vi "drive-auto.vi"() -> ()   [LabVIEW 2018]
doc: "This VI is called for each TeleOp packet received from the DS where the robot is not disabled. It is often used to read from the joysticks and update I/O or to update setpoints for timed control loops. It should complete and return within 20 milliseconds or it may miss DS packets."
uses:
  <vilib>/Rock Robotics/WPI/Solenoid/WPI_SolenoidValue.ctl
  <vilib>/Rock Robotics/WPI/ThirdParty/Phoenix-LabVIEW/Motor Controller/Controls/CTRE_Phoenix_MotorControl_ControlMode.ctl
  069bde93-6a50-4702-a448-63a100da85ba.vi
  93fe4f39-d887-44e8-b42b-40b0db67de57.vi
  <vilib>/Rock Robotics/WPI/Utilities/WPI_GetSetVariantRefNum.vi
  <vilib>/Rock Robotics/Network Tables/NT Write Boolean Array.vi
  <vilib>/Rock Robotics/Network Tables/NT Write Numeric Array.vi
  Robot Global Data.vi
  <vilib>/Rock Robotics/WPI/Solenoid/WPI_SolenoidSetEnum.vi
  <vilib>/Rock Robotics/WPI/ThirdParty/Phoenix-LabVIEW/Motor Controller/Get/CTRE_Phoenix_MotorController_GetSelectedSensorData.vi
  <vilib>/Rock Robotics/WPI/ThirdParty/Phoenix-LabVIEW/Motor Controller/Get/CTRE_Phoenix_MotorController_GetOutputCurrent_Enhanced.vi
panel:
  out "Level":string="Low"
  out "GamePiece":string="Hatch"
  out "Output Voltage 4":dbl
  out "Output Voltage 3":dbl
  out "Output Voltage 2":dbl
  out "Output Voltage":dbl
  out "wrist sensor":i32
  out "Arm sensor":i32
  out "x output 2":dbl
  out "y output 2":dbl
  # "left"
  # "RIGHT"
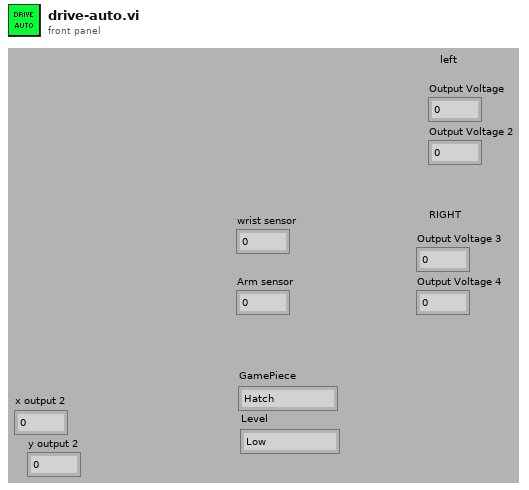
[diagram p1: front panel]
types:
  T1 = typedef "WPI_SolenoidValue.ctl" = enum16{"Off", "On", "Forward", "Reverse"}
  T2 = typedef "WPI_JoystickDevRef.ctl" = cluster{"Device":T3}
  T3 = typedef "WPI_JoystickDeviceEnum.ctl" = enum16{"USB 0", "USB 1", "USB 2", "USB 3", "USB 4", "USB 5"}
  T4 = typedef "WPI_RobotDriveDevRef.ctl" = cluster{"DevStatus":errorcluster, "Motors[]":T5[], "Square Inputs":bool, "Max Output":dbl}
  T5 = typedef "WPI_MotorControlDeviceRef.ctl" = cluster{"DeviceStatus":errorcluster, "Type":T6, "PWM":cluster{"PWM Channel":T7, "DeadBand":T8}, "CAN":cluster{"Device Number":u8, "SetOutput VI Ref":variant, "GetOutput VI Ref":variant, "Enable VI Ref":variant, "Disable VI Ref":variant, "Data":variant}, "Invert":bool, "DIO PWM":cluster{"PWM \"Enable\" Channel":T7, "DIOChannel":T9, "PWM Rate":dbl}}
  T6 = typedef "WPI_MotorControlType.ctl" = enum16{"PWM", "CAN", "DIO PWM"}
  T7 = typedef "FPGA_DIOPWMChannel.ctl" = enum8{"PWM 0", "PWM 1", "PWM 2", "PWM 3", "PWM 4", "PWM 5", "PWM 6", "PWM 7", "PWM 8", "PWM 9", "PWM MXP 0", "PWM MXP 1", "PWM MXP 2", "PWM MXP 3", "PWM MXP 4", "PWM MXP 5", "PWM MXP 6", "PWM MXP 7", "PWM MXP 8", "PWM MXP 9", "Invalid"}
  T8 = typedef "WPI_PWMDeadband.ctl" = cluster{"Name":string, "maxPositivePwm":i32, "minPositivePwm":i32, "centerPwm":i32, "maxNegativePwm":i32, "minNegativePwm":i32, "angularRange":u16}
  T9 = typedef "FPGA_DIOChannel.ctl" = enum8{"DIO 0", "DIO 1", "DIO 2", "DIO 3", "DIO 4", "DIO 5", "DIO 6", "DIO 7", "DIO 8", "DIO 9", "DIO MXP 0", "DIO MXP 1", "DIO MXP 2", "DIO MXP 3", "DIO MXP 4", "DIO MXP 5", "DIO MXP 6", "DIO MXP 7", "DIO MXP 8", "DIO MXP 9", "DIO MXP 10", "DIO MXP 11", "DIO MXP 12", "DIO MXP 13", "DIO MXP 14", "DIO MXP 15", "SPI Port CS1", "SPI Port CS2", "SPI Port CS3", "SPI Port MISO", "SPI Port MOSI", "Invalid"}
  T10 = typedef "WPI_SolenoidDevRef.ctl" = cluster{"DevStatus":errorcluster, "Pneumatics Control Module":u8, "Forward Solenoid Channel":T11, "Reverse Solenoid Channel":T11}
  T11 = typedef "WPI_SolenoidChannel.ctl" = enum8{"Solenoid 0", "Solenoid 1", "Solenoid 2", "Solenoid 3", "Solenoid 4", "Solenoid 5", "Solenoid 6", "Solenoid 7", "Invalid"}
  T12 = typedef "CTRE_Phoenix_MotorControl_ControlMode.ctl" = u16
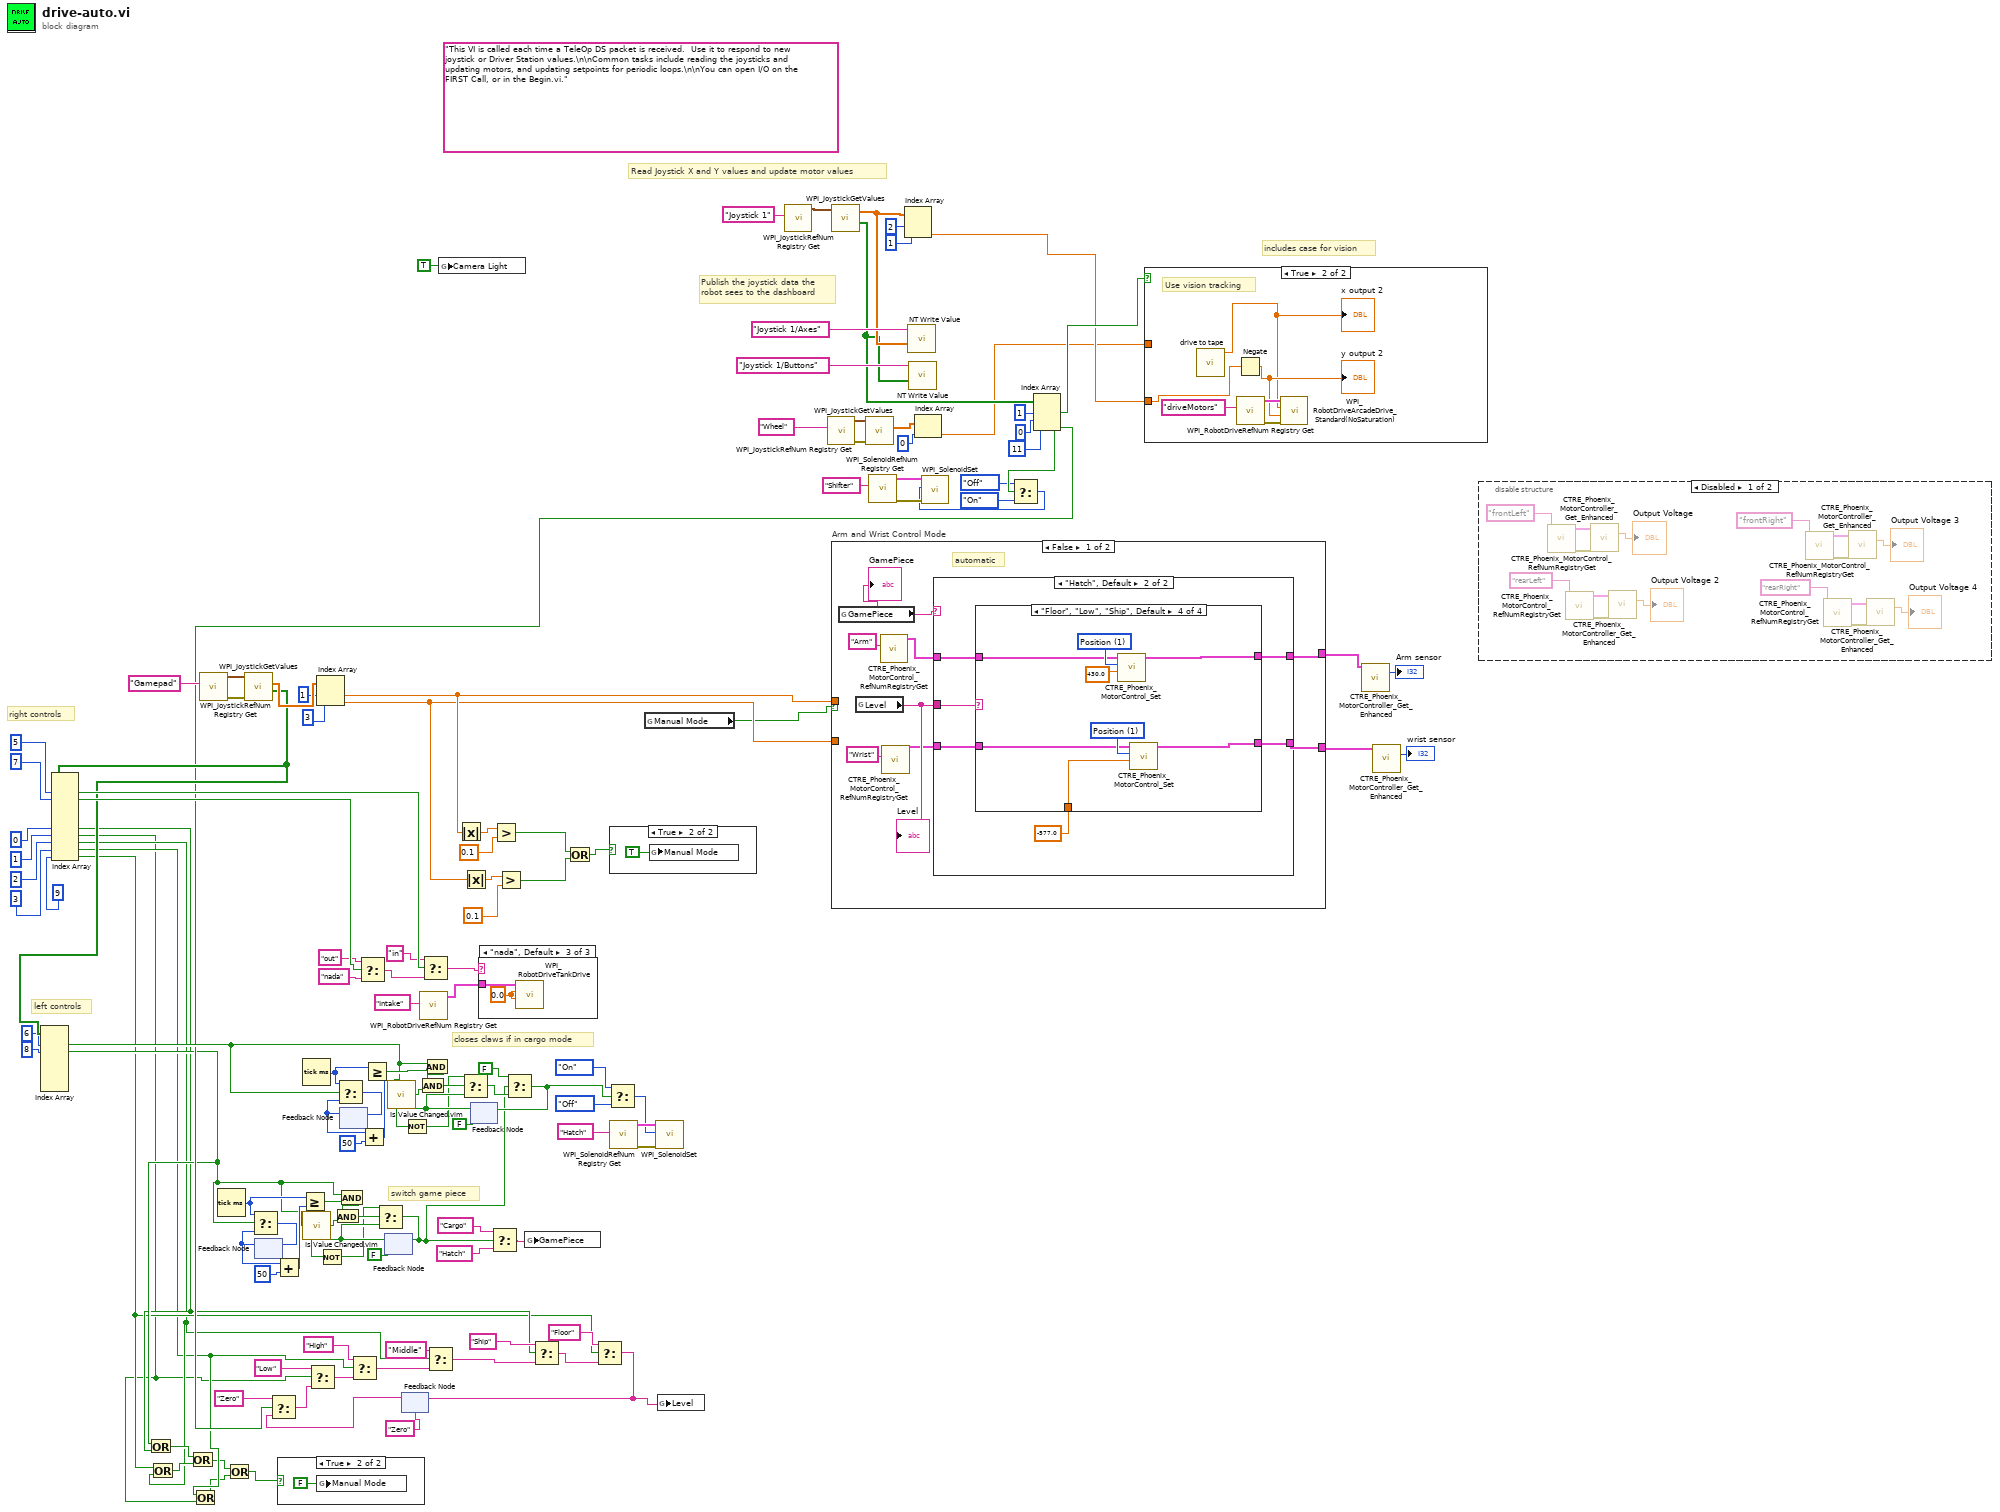
[diagram p0: block diagram]
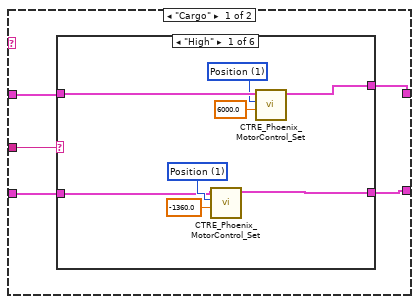
[diagram p5: hidden frame]
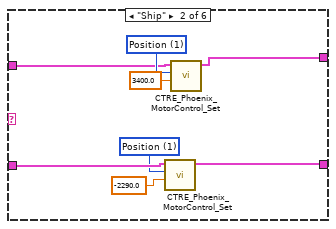
[diagram p6: hidden frame]
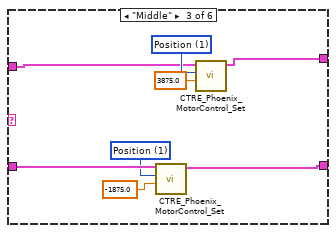
[diagram p7: hidden frame]
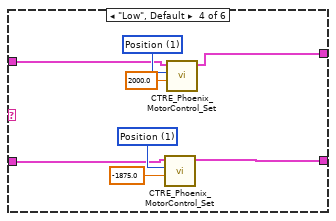
[diagram p8: hidden frame]
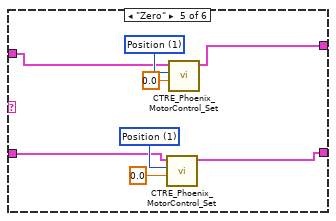
[diagram p9: hidden frame]
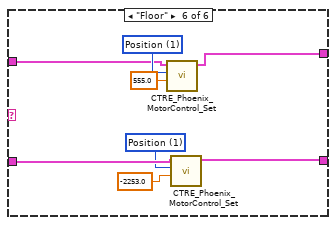
[diagram p10: hidden frame]
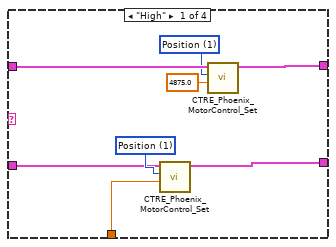
[diagram p11: hidden frame]
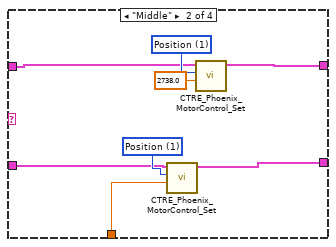
[diagram p12: hidden frame]
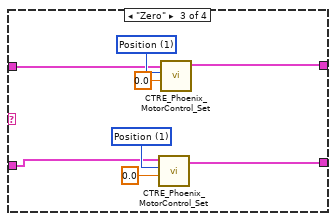
[diagram p13: hidden frame]
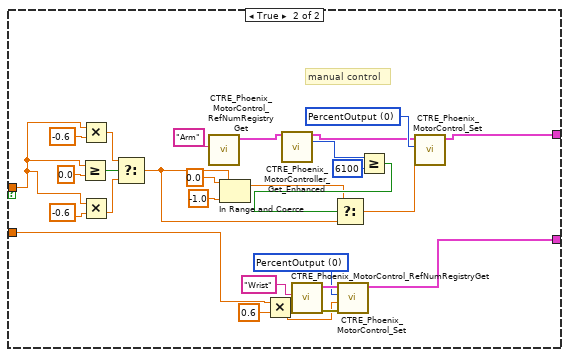
[diagram p14: hidden frame]
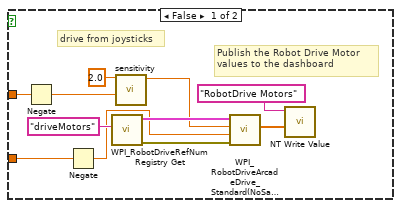
[diagram p15: hidden frame]
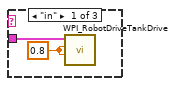
[diagram p16: hidden frame]
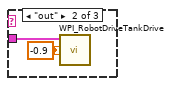
[diagram p17: hidden frame]
diagram:
  (unwired) "This VI is called each time a TeleOp DS packet is received.  Use it to respond to new joystick or Driver Station values.\n\nCommon tasks include reading the joysticks and updating motors, and updating setpoints for periodic loops.\n\nYou can open I/O on the FIRST Call, or in the Begin.vi."
  # "closes claws if in cargo mode"
  # "switch game piece"
  # "left controls"
  # "right controls"
  # "includes case for vision"
  # "Publish the joystick data the\nrobot sees to the dashboard"
  # "Read Joystick X and Y values and update motor values"
  n1 = call <vilib>:"WPI_JoystickRefNum Registry Get.vi"("refnum name"="Gamepad") -> ("error out"=w112:errorcluster, "JoystickDevRef"=w115:T2)  [unwired: 1 in, 8 out]
  n2 = Tick Count (ms)() -> (millisecond timer value=w62:u32)
  n3 = call <vilib>:"WPI_JoystickGetValues.vi"("error in (no error)"=w112, "JoystickDevRef"=w115) -> ("Buttons"=w36:bool[], "Axes"=w114:dbl[])  [unwired: 5 in, 3 out]
  n4 = Index Array(array=w36, index #1=6 ("index"), index #2=8 ("index")) -> (element #1=w33:bool, element #2=w9:bool)  [unwired: 5 in, 5 out]
  n5 = Index Array(array=w36, index #1=5 ("index"), index #2=7 ("index"), index #6=0 ("index"), index #7=1 ("index"), index #8=2 ("index"), index #9=3 ("index"), index #10=9 ("index")) -> (element #1=w109:bool, element #2=w104:bool, element #6=w8:bool, element #7=w4:bool, element #8=w6:bool, element #9=w5:bool, element #10=w7:bool)  [unwired: 3 in, 3 out]
  n6 = Or(x=w9, y=w8) -> (x .or. y?=w11:bool)
  n7 = Or(x=w7, y=w6) -> (x .or. y?=w10:bool)
  n8 = Or(x=w11, y=w10) -> (x .or. y?=w2:bool)
  n9 = Or(x=w5, y=w4) -> (x .or. y?=w3:bool)
  n10 = Or(x=w2, y=w3) -> (x .or. y?=w1:bool)
  n11 = feedback #1() -> (w53:u32)  [unwired: 1 in]
  n12 = Select(t=w62, s=w9, f=w53) -> (s? t:f=w60:u32)
  n13 = feedback-in #1(w60) -> ()
  n14 = Add(x=w53, y=u32 50) -> (x+y=w61:u32)
  n15 = case shown="True" w1 {
    frame False {
    }
    frame True {
      n16 = global write "Robot Global Data.vi" "Manual Mode"(FALSE) -> ()
    }
  }
  n17 = Greater Or Equal?(x=w62, y=w61) -> (x >= y?=w63:bool)
  n18 = Tick Count (ms)() -> (millisecond timer value=w79:u32)
  n19 = call "Is Value Changed.vim"("value"=w9) -> ("changed or first call?"=w58:bool)
  n20 = Index Array(array=w114, index #1=1 ("index"), index #2=3 ("index")) -> (element #1=w20:dbl, element #2=w15:dbl)
  n21 = And(x=w9, y=w63) -> (x .and. y?=w64:bool)
  n22 = And(x=w64, y=w58) -> (x .and. y?=w57:bool)
  n23 = feedback #2() -> (w70:u32)  [unwired: 1 in]
  n24 = Select(t=w79, s=w33, f=w70) -> (s? t:f=w77:u32)
  n25 = feedback-in #2(w77) -> ()
  n26 = Select(t="out", s=w104, f="nada") -> (s? t:f=w105:string)
  n27 = Add(x=w70, y=u32 50) -> (x+y=w78:u32)
  n28 = Greater Or Equal?(x=w79, y=w78) -> (x >= y?=w80:bool)
  n29 = feedback #3(FALSE) -> (w56:bool)
  n30 = Not(x=w56) -> (.not. x?=w54:bool)
  n31 = Select(t=w54, s=w57, f=w56) -> (s? t:f=w24:bool)
  n32 = feedback-in #3(w24) -> ()
  n33 = call "Is Value Changed.vim"("value"=w33) -> ("changed or first call?"=w75:bool)
  n34 = feedback #4("Zero") -> (w30:string)
  n35 = call <vilib>:"WPI_RobotDriveRefNum Registry Get.vi"("refnum name"="Intake") -> ("RobotDriveDevRef"=w100:T4)  [unwired: 9 in, 1 out]
  n36 = Select(t="in", s=w109, f=w105) -> (s? t:f=w108:string)
  n37 = And(x=w33, y=w80) -> (x .and. y?=w81:bool)
  n38 = And(x=w81, y=w75) -> (x .and. y?=w74:bool)
  n39 = global write "Robot Global Data.vi" "Camera Light"(TRUE ("Camera Light")) -> ()
  n40 = Absolute Value(x=w20) -> (abs(x)=w22:dbl)
  n41 = Absolute Value(x=w15) -> (abs(x)=w18:dbl)
  n42 = feedback #5(FALSE) -> (w73:bool)
  n43 = Not(x=w73) -> (.not. x?=w71:bool)
  n44 = Select(t=w71, s=w74, f=w73) -> (s? t:f=w25:bool)
  n45 = case shown="\"nada\", Default" w108 {
    tunnel: w100 -> [w132 w134 w136]
    frame "in" {
      w133 = 0.8
      n46 = call <vilib>:"WPI_RobotDriveTankDrive.vi"("Right axis value"=w133, "Left axis value"=w133, "RobotDriveDevRef"=w132) -> ()  [unwired: 6 in, 3 out]
    }
    frame "out" {
      w135 = -0.9
      n47 = call <vilib>:"WPI_RobotDriveTankDrive.vi"("Right axis value"=w135, "Left axis value"=w135, "RobotDriveDevRef"=w134) -> ()  [unwired: 6 in, 3 out]
    }
    frame "nada", Default {
      w137 = 0.0
      n48 = call <vilib>:"WPI_RobotDriveTankDrive.vi"("Right axis value"=w137, "Left axis value"=w137, "RobotDriveDevRef"=w136) -> ()  [unwired: 6 in, 3 out]
    }
  }
  n49 = Select(t="Cargo", s=w24, f="Hatch") -> (s? t:f=w66:string)
  n50 = Greater?(x=w22, y=0.1) -> (0:w19:bool)
  n51 = Greater?(x=w18, y=0.1) -> (0:w16:bool)
  n52 = Select(t=FALSE, s=w24, f=w25) -> (s? t:f=w26:bool)
  n53 = feedback-in #5(w26) -> ()
  n54 = global write "Robot Global Data.vi" "GamePiece"(w66) -> ()
  n55 = Or(x=w19, y=w16) -> (x .or. y?=w13:bool)
  n56 = Select(t=WPI_SolenoidValue."On" ("Value"), s=w26, f=WPI_SolenoidValue."Off") -> (s? t:f=w96:T1)
  n57 = case shown="True" w13 {
    frame False {
    }
    frame True {
      n58 = global write "Robot Global Data.vi" "Manual Mode"(TRUE) -> ()
    }
  }
  n59 = call <vilib>:"WPI_SolenoidRefNum Registry Get.vi"("refnum name"="Hatch") -> ("error out"=w99:errorcluster, "SolenoidDevRef"=w98:T10)  [unwired: 9 in]
  n60 = global read "Robot Global Data.vi" "Manual Mode"() -> (w14:bool)
  n61 = call-poly <vilib>:"WPI_SolenoidSet.vi"("error in (no error)"=w99, "Value"=w96, "SolenoidDevRef"=w98) -> ()  [unwired: 7 in, 2 out]
  n62 = call <vilib>:"WPI_JoystickRefNum Registry Get.vi"("refnum name"="Joystick 1") -> ("JoystickDevRef"=w129:T2)  [unwired: 1 in, 9 out]
  n63 = call <vilib>:"WPI_JoystickRefNum Registry Get.vi"("refnum name"="Wheel") -> ("error out"=w123:errorcluster, "JoystickDevRef"=w122:T2)  [unwired: 9 in]
  n64 = call <vilib>:"WPI_JoystickGetValues.vi"("JoystickDevRef"=w129) -> ("Buttons"=w118:bool[], "Axes"=w126:dbl[])  [unwired: 6 in, 3 out]
  n65 = case "Arm and Wrist Control Mode" shown="False" w14 {
    tunnel: w15 -> [_ w258]
    tunnel: w20 -> [_ w250]
    tunnel: [w139 w249] -> w68
    tunnel: [w143 w248] -> w67
    frame False {
      # "automatic"
      n66 = global read "Robot Global Data.vi" "GamePiece"() -> (w142:string)
      "GamePiece" <- w142
      n67 = global read "Robot Global Data.vi" "Level"() -> (w141:string)
      "Level" <- w141
      n68 = call <vilib>:"CTRE_Phoenix_MotorControl_RefNumRegistryGet.vi"("refnum name"="Arm") -> ("PhoenixMotorControlDevRef"=w146:T5)  [unwired: 9 in, 1 out]
      n69 = call <vilib>:"CTRE_Phoenix_MotorControl_RefNumRegistryGet.vi"("refnum name"="Wrist") -> ("PhoenixMotorControlDevRef"=w140:T5)  [unwired: 9 in, 1 out]
      n70 = case shown="\"Hatch\", Default" w142 {
        tunnel: w146 -> [w150 w205]
        tunnel: [w151 w204] -> w143
        tunnel: [w149 w203] -> w139
        tunnel: w141 -> [w148 w202]
        tunnel: w140 -> [w147 w201]
        frame "Cargo" {
          n71 = case shown="\"High\"" w148 {
            tunnel: w150 -> [w159 w166 w174 w182 w187 w198]
            tunnel: [w157 w165 w173 w181 w186 w197] -> w151
            tunnel: [w155 w163 w171 w179 w185 w195] -> w149
            tunnel: w147 -> [w152 w162 w170 w176 w184 w194]
            frame "High" {
              w153 = T12 1 items=["PercentOutput"=0, "Position"=1, "Velocity"=2, "Current"=3, "Follower"=5, "MotionProfile"=6, "MotionMagic"=7, "MotionProfileArc"=10, "Disabled"=15] ("Control Mode")
              w158 = T12 1 items=["PercentOutput"=0, "Position"=1, "Velocity"=2, "Current"=3, "Follower"=5, "MotionProfile"=6, "MotionMagic"=7, "MotionProfileArc"=10, "Disabled"=15] ("Control Mode")
              n72 = call <vilib>:"CTRE_Phoenix_MotorControl_Set.vi"("Output"=-1360.0, "Control Mode"=w153, "PhoenixMotorControlDevRef"=w152) -> ("PhoenixMotorControlDevRef"=w155:T5)  [unwired: 7 in, 1 out]
              n73 = call <vilib>:"CTRE_Phoenix_MotorControl_Set.vi"("Output"=6000.0, "Control Mode"=w158, "PhoenixMotorControlDevRef"=w159) -> ("PhoenixMotorControlDevRef"=w157:T5)  [unwired: 7 in, 1 out]
            }
            frame "Ship" {
              w160 = T12 1 items=["PercentOutput"=0, "Position"=1, "Velocity"=2, "Current"=3, "Follower"=5, "MotionProfile"=6, "MotionMagic"=7, "MotionProfileArc"=10, "Disabled"=15] ("Control Mode")
              w167 = T12 1 items=["PercentOutput"=0, "Position"=1, "Velocity"=2, "Current"=3, "Follower"=5, "MotionProfile"=6, "MotionMagic"=7, "MotionProfileArc"=10, "Disabled"=15] ("Control Mode")
              n74 = call <vilib>:"CTRE_Phoenix_MotorControl_Set.vi"("Output"=-2290.0, "Control Mode"=w160, "PhoenixMotorControlDevRef"=w162) -> ("PhoenixMotorControlDevRef"=w163:T5)  [unwired: 7 in, 1 out]
              n75 = call <vilib>:"CTRE_Phoenix_MotorControl_Set.vi"("Output"=3400.0, "Control Mode"=w167, "PhoenixMotorControlDevRef"=w166) -> ("PhoenixMotorControlDevRef"=w165:T5)  [unwired: 7 in, 1 out]
            }
            frame "Middle" {
              w168 = T12 1 items=["PercentOutput"=0, "Position"=1, "Velocity"=2, "Current"=3, "Follower"=5, "MotionProfile"=6, "MotionMagic"=7, "MotionProfileArc"=10, "Disabled"=15] ("Control Mode")
              w175 = T12 1 items=["PercentOutput"=0, "Position"=1, "Velocity"=2, "Current"=3, "Follower"=5, "MotionProfile"=6, "MotionMagic"=7, "MotionProfileArc"=10, "Disabled"=15] ("Control Mode")
              n76 = call <vilib>:"CTRE_Phoenix_MotorControl_Set.vi"("Output"=-1875.0, "Control Mode"=w168, "PhoenixMotorControlDevRef"=w170) -> ("PhoenixMotorControlDevRef"=w171:T5)  [unwired: 7 in, 1 out]
              n77 = call <vilib>:"CTRE_Phoenix_MotorControl_Set.vi"("Output"=3875.0, "Control Mode"=w175, "PhoenixMotorControlDevRef"=w174) -> ("PhoenixMotorControlDevRef"=w173:T5)  [unwired: 7 in, 1 out]
            }
            frame "Low", Default {
              w177 = T12 1 items=["PercentOutput"=0, "Position"=1, "Velocity"=2, "Current"=3, "Follower"=5, "MotionProfile"=6, "MotionMagic"=7, "MotionProfileArc"=10, "Disabled"=15] ("Control Mode")
              w183 = T12 1 items=["PercentOutput"=0, "Position"=1, "Velocity"=2, "Current"=3, "Follower"=5, "MotionProfile"=6, "MotionMagic"=7, "MotionProfileArc"=10, "Disabled"=15] ("Control Mode")
              n78 = call <vilib>:"CTRE_Phoenix_MotorControl_Set.vi"("Output"=-1875.0, "Control Mode"=w177, "PhoenixMotorControlDevRef"=w176) -> ("PhoenixMotorControlDevRef"=w179:T5)  [unwired: 7 in, 1 out]
              n79 = call <vilib>:"CTRE_Phoenix_MotorControl_Set.vi"("Output"=2000.0, "Control Mode"=w183, "PhoenixMotorControlDevRef"=w182) -> ("PhoenixMotorControlDevRef"=w181:T5)  [unwired: 7 in, 1 out]
            }
            frame "Zero" {
              w188 = T12 1 items=["PercentOutput"=0, "Position"=1, "Velocity"=2, "Current"=3, "Follower"=5, "MotionProfile"=6, "MotionMagic"=7, "MotionProfileArc"=10, "Disabled"=15] ("Control Mode")
              w191 = T12 1 items=["PercentOutput"=0, "Position"=1, "Velocity"=2, "Current"=3, "Follower"=5, "MotionProfile"=6, "MotionMagic"=7, "MotionProfileArc"=10, "Disabled"=15] ("Control Mode")
              n80 = call <vilib>:"CTRE_Phoenix_MotorControl_Set.vi"("Output"=0.0, "Control Mode"=w188, "PhoenixMotorControlDevRef"=w184) -> ("PhoenixMotorControlDevRef"=w185:T5)  [unwired: 7 in, 1 out]
              n81 = call <vilib>:"CTRE_Phoenix_MotorControl_Set.vi"("Output"=0.0, "Control Mode"=w191, "PhoenixMotorControlDevRef"=w187) -> ("PhoenixMotorControlDevRef"=w186:T5)  [unwired: 7 in, 1 out]
            }
            frame "Floor" {
              w192 = T12 1 items=["PercentOutput"=0, "Position"=1, "Velocity"=2, "Current"=3, "Follower"=5, "MotionProfile"=6, "MotionMagic"=7, "MotionProfileArc"=10, "Disabled"=15] ("Control Mode")
              w199 = T12 1 items=["PercentOutput"=0, "Position"=1, "Velocity"=2, "Current"=3, "Follower"=5, "MotionProfile"=6, "MotionMagic"=7, "MotionProfileArc"=10, "Disabled"=15] ("Control Mode")
              n82 = call <vilib>:"CTRE_Phoenix_MotorControl_Set.vi"("Output"=555.0, "Control Mode"=w199, "PhoenixMotorControlDevRef"=w198) -> ("PhoenixMotorControlDevRef"=w197:T5)  [unwired: 7 in, 1 out]
              n83 = call <vilib>:"CTRE_Phoenix_MotorControl_Set.vi"("Output"=-2253.0, "Control Mode"=w192, "PhoenixMotorControlDevRef"=w194) -> ("PhoenixMotorControlDevRef"=w195:T5)  [unwired: 7 in, 1 out]
            }
          }
        }
        frame "Hatch", Default {
          n84 = case shown="\"Floor\", \"Low\", \"Ship\", Default" w202 {
            tunnel: w205 -> [w213 w220 w225 w236]
            tunnel: [w211 w219 w224 w235] -> w204
            tunnel: [w209 w217 w223 w233] -> w203
            tunnel: w201 -> [w207 w215 w222 w231]
            tunnel: -577.0 ("Output") -> [w206 w214 _ w230]
            frame "High" {
              w208 = T12 1 items=["PercentOutput"=0, "Position"=1, "Velocity"=2, "Current"=3, "Follower"=5, "MotionProfile"=6, "MotionMagic"=7, "MotionProfileArc"=10, "Disabled"=15] ("Control Mode")
              w212 = T12 1 items=["PercentOutput"=0, "Position"=1, "Velocity"=2, "Current"=3, "Follower"=5, "MotionProfile"=6, "MotionMagic"=7, "MotionProfileArc"=10, "Disabled"=15] ("Control Mode")
              n85 = call <vilib>:"CTRE_Phoenix_MotorControl_Set.vi"("Output"=w206, "Control Mode"=w208, "PhoenixMotorControlDevRef"=w207) -> ("PhoenixMotorControlDevRef"=w209:T5)  [unwired: 7 in, 1 out]
              n86 = call <vilib>:"CTRE_Phoenix_MotorControl_Set.vi"("Output"=4875.0, "Control Mode"=w212, "PhoenixMotorControlDevRef"=w213) -> ("PhoenixMotorControlDevRef"=w211:T5)  [unwired: 7 in, 1 out]
            }
            frame "Middle" {
              w216 = T12 1 items=["PercentOutput"=0, "Position"=1, "Velocity"=2, "Current"=3, "Follower"=5, "MotionProfile"=6, "MotionMagic"=7, "MotionProfileArc"=10, "Disabled"=15] ("Control Mode")
              w221 = T12 1 items=["PercentOutput"=0, "Position"=1, "Velocity"=2, "Current"=3, "Follower"=5, "MotionProfile"=6, "MotionMagic"=7, "MotionProfileArc"=10, "Disabled"=15] ("Control Mode")
              n87 = call <vilib>:"CTRE_Phoenix_MotorControl_Set.vi"("Output"=w214, "Control Mode"=w216, "PhoenixMotorControlDevRef"=w215) -> ("PhoenixMotorControlDevRef"=w217:T5)  [unwired: 7 in, 1 out]
              n88 = call <vilib>:"CTRE_Phoenix_MotorControl_Set.vi"("Output"=2738.0, "Control Mode"=w221, "PhoenixMotorControlDevRef"=w220) -> ("PhoenixMotorControlDevRef"=w219:T5)  [unwired: 7 in, 1 out]
            }
            frame "Zero" {
              w226 = T12 1 items=["PercentOutput"=0, "Position"=1, "Velocity"=2, "Current"=3, "Follower"=5, "MotionProfile"=6, "MotionMagic"=7, "MotionProfileArc"=10, "Disabled"=15] ("Control Mode")
              w229 = T12 1 items=["PercentOutput"=0, "Position"=1, "Velocity"=2, "Current"=3, "Follower"=5, "MotionProfile"=6, "MotionMagic"=7, "MotionProfileArc"=10, "Disabled"=15] ("Control Mode")
              n89 = call <vilib>:"CTRE_Phoenix_MotorControl_Set.vi"("Output"=0.0, "Control Mode"=w226, "PhoenixMotorControlDevRef"=w222) -> ("PhoenixMotorControlDevRef"=w223:T5)  [unwired: 7 in, 1 out]
              n90 = call <vilib>:"CTRE_Phoenix_MotorControl_Set.vi"("Output"=0.0, "Control Mode"=w229, "PhoenixMotorControlDevRef"=w225) -> ("PhoenixMotorControlDevRef"=w224:T5)  [unwired: 7 in, 1 out]
            }
            frame "Floor", "Low", "Ship", Default {
              w232 = T12 1 items=["PercentOutput"=0, "Position"=1, "Velocity"=2, "Current"=3, "Follower"=5, "MotionProfile"=6, "MotionMagic"=7, "MotionProfileArc"=10, "Disabled"=15] ("Control Mode")
              w237 = T12 1 items=["PercentOutput"=0, "Position"=1, "Velocity"=2, "Current"=3, "Follower"=5, "MotionProfile"=6, "MotionMagic"=7, "MotionProfileArc"=10, "Disabled"=15] ("Control Mode")
              n91 = call <vilib>:"CTRE_Phoenix_MotorControl_Set.vi"("Output"=430.0, "Control Mode"=w237, "PhoenixMotorControlDevRef"=w236) -> ("PhoenixMotorControlDevRef"=w235:T5)  [unwired: 7 in, 1 out]
              n92 = call <vilib>:"CTRE_Phoenix_MotorControl_Set.vi"("Output"=w230, "Control Mode"=w232, "PhoenixMotorControlDevRef"=w231) -> ("PhoenixMotorControlDevRef"=w233:T5)  [unwired: 7 in, 1 out]
            }
          }
        }
      }
    }
    frame True {
      w261 = T12 0 items=["PercentOutput"=0, "Position"=1, "Velocity"=2, "Current"=3, "Follower"=5, "MotionProfile"=6, "MotionMagic"=7, "MotionProfileArc"=10, "Disabled"=15] ("Control Mode")
      w265 = T12 0 items=["PercentOutput"=0, "Position"=1, "Velocity"=2, "Current"=3, "Follower"=5, "MotionProfile"=6, "MotionMagic"=7, "MotionProfileArc"=10, "Disabled"=15] ("Control Mode")
      # "manual control"
      n93 = Greater Or Equal?(x=w250, y=0.0) -> (x >= y?=w256:bool)
      n94 = Multiply(x=w250, y=-0.6) -> (x*y=w251:dbl)
      n95 = Multiply(x=w250, y=-0.6) -> (x*y=w255:dbl)
      n96 = Select(t=w251, s=w256, f=w255) -> (s? t:f=w242:dbl)
      n97 = call <vilib>:"CTRE_Phoenix_MotorControl_RefNumRegistryGet.vi"("refnum name"="Arm") -> ("PhoenixMotorControlDevRef"=w246:T5)  [unwired: 9 in, 1 out]
      n98 = In Range and Coerce(upper limit=0.0, x=w242, lower limit=-1.0) -> (coerced(x)=w238:dbl)  [unwired: 1 out]
      n99 = Multiply(x=w258, y=0.6) -> (x*y=w259:dbl)
      n100 = call-poly <vilib>:"CTRE_Phoenix_MotorController_Get_Enhanced.vi"("PhoenixMotorControlDevRef"=w246) -> ("PhoenixMotorControlDevRef"=w247:T5, "Position (Raw Sensor Units)"=w245:i32)  [unwired: 11 in, 2 out]
      n101 = call <vilib>:"CTRE_Phoenix_MotorControl_RefNumRegistryGet.vi"("refnum name"="Wrist") -> ("error out"=w263:errorcluster, "PhoenixMotorControlDevRef"=w262:T5)  [unwired: 9 in]
      n102 = call <vilib>:"CTRE_Phoenix_MotorControl_Set.vi"("error in (no error)"=w263, "Output"=w259, "Control Mode"=w261, "PhoenixMotorControlDevRef"=w262) -> ("PhoenixMotorControlDevRef"=w249:T5)  [unwired: 6 in, 1 out]
      n103 = Greater Or Equal?(x=w245, y=6100) -> (x >= y?=w243:bool)
      n104 = Select(t=w238, s=w243, f=w242) -> (s? t:f=w239:dbl)
      n105 = call <vilib>:"CTRE_Phoenix_MotorControl_Set.vi"("Output"=w239, "Control Mode"=w265, "PhoenixMotorControlDevRef"=w247) -> ("PhoenixMotorControlDevRef"=w248:T5)  [unwired: 7 in, 1 out]
    }
  }
  n106 = call <vilib>:"WPI_JoystickGetValues.vi"("error in (no error)"=w123, "JoystickDevRef"=w122) -> ("Axes"=w121:dbl[])  [unwired: 5 in, 4 out]
  n107 = call <vilib>:"WPI_SolenoidRefNum Registry Get.vi"("refnum name"="Shifter") -> ("error out"=w92:errorcluster, "SolenoidDevRef"=w91:T10)  [unwired: 9 in]
  n108 = Index Array(array=w126, index #1=2 ("index"), index #2=1 ("index")) -> (element #2=w83:dbl)  [unwired: 1 out]
  n109 = call-poly <vilib>:"NT Write Value.vi"("Numeric Array"=w126, "Name"="Joystick 1/Axes") -> ()  [unwired: 9 in, 1 out]
  n110 = call-poly <vilib>:"NT Write Value.vi"("Boolean Array"=w118, "Name"="Joystick 1/Buttons") -> ()  [unwired: 9 in, 1 out]
  n111 = Index Array(array=w121, index=0) -> (element=w82:dbl)
  n112 = Index Array(array=w118, index #1=1 ("index"), index #2=0 ("index"), index #3=11 ("index")) -> (element #1=w84:bool, element #2=w89:bool, element #3=w12:bool)
  n113 = Select(t="Zero", s=w12, f=w30) -> (s? t:f=w27:string)
  n114 = Select(t="Low", s=w4, f=w27) -> (s? t:f=w44:string)
  n115 = Select(t="High", s=w5, f=w44) -> (s? t:f=w43:string)
  n116 = Select(t="Middle", s=w6, f=w43) -> (s? t:f=w41:string)
  n117 = Select(t="Ship", s=w8, f=w41) -> (s? t:f=w37:string)
  n118 = Select(t="Floor", s=w7, f=w37) -> (s? t:f=w39:string)
  n119 = feedback-in #4(w39) -> ()
  n120 = global write "Robot Global Data.vi" "Level"(w39) -> ()
  n121 = Select(t=WPI_SolenoidValue."Off" ("Value"), s=w89, f=WPI_SolenoidValue."On" ("Value")) -> (s? t:f=w88:T1)
  n122 = call-poly <vilib>:"WPI_SolenoidSet.vi"("error in (no error)"=w92, "Value"=w88, "SolenoidDevRef"=w91) -> ()  [unwired: 7 in, 2 out]
  n123 = case shown="True" w84 {
    tunnel: w83 -> [w272 w277]
    tunnel: w82 -> [w271 _]
    frame False {
      # "drive from joysticks"
      # "Publish the Robot Drive Motor\nvalues to the dashboard"
      n124 = Negate(x=w271) -> (-x=w268:dbl)
      n125 = Negate(x=w272) -> (-x=w269:dbl)
      n126 = call <vilib>:"WPI_RobotDriveRefNum Registry Get.vi"("refnum name"="driveMotors") -> ("error out"=w270:errorcluster, "RobotDriveDevRef"=w275:T4)  [unwired: 1 in, 8 out]
      n127 = call "sensitivity.vi"("x"=w268, "sensitivity"=2.0) -> ("scaled value"=w267:dbl)  [unwired: 9 in]
      n128 = call <vilib>:"WPI_RobotDriveArcadeDrive_Standard(NoSaturation).vi"("error in (no error)"=w270, "Y axis value"=w269, "X axis value"=w267, "RobotDriveDevRef"=w275) -> ("Motor Values"=w276:dbl[])  [unwired: 7 out]
      n129 = call-poly <vilib>:"NT Write Value.vi"("Numeric Array"=w276, "Name"="RobotDrive Motors") -> ()  [unwired: 9 in, 1 out]
    }
    frame True {
      # "Use vision tracking"
      n130 = call "drive to tape.vi"() -> ("x output"=w278:dbl)  [unwired: 10 in, 1 out]
      "x output 2" <- w278
      n131 = Negate(x=w277) -> (-x=w279:dbl)
      "y output 2" <- w279
      n132 = call <vilib>:"WPI_RobotDriveRefNum Registry Get.vi"("refnum name"="driveMotors") -> ("error out"=w280:errorcluster, "RobotDriveDevRef"=w281:T4)  [unwired: 1 in, 8 out]
      n133 = call <vilib>:"WPI_RobotDriveArcadeDrive_Standard(NoSaturation).vi"("error in (no error)"=w280, "Y axis value"=w279, "X axis value"=w278, "RobotDriveDevRef"=w281) -> ()  [unwired: 8 out]
    }
  }
  n134 = call-poly <vilib>:"CTRE_Phoenix_MotorController_Get_Enhanced.vi"("PhoenixMotorControlDevRef"=w67) -> ("Position (Raw Sensor Units)"=→"Arm sensor":i32)  [unwired: 11 in, 3 out]
  n135 = call-poly <vilib>:"CTRE_Phoenix_MotorController_Get_Enhanced.vi"("PhoenixMotorControlDevRef"=w68) -> ("Position (Raw Sensor Units)"=→"wrist sensor":i32)  [unwired: 11 in, 3 out]
  n136 = disable-structure shown="Disabled" {
    frame Disabled {
      n137 = call <vilib>:"CTRE_Phoenix_MotorControl_RefNumRegistryGet.vi"("refnum name"="frontLeft") -> ("error out"=w297:errorcluster, "PhoenixMotorControlDevRef"=w298:T5)  [unwired: 9 in]
      n138 = call <vilib>:"CTRE_Phoenix_MotorControl_RefNumRegistryGet.vi"("refnum name"="rearLeft") -> ("error out"=w294:errorcluster, "PhoenixMotorControlDevRef"=w295:T5)  [unwired: 9 in]
      n139 = call-poly <vilib>:"CTRE_Phoenix_MotorController_Get_Enhanced.vi"("PhoenixMotorControlDevRef"=w298, "error in"=w297) -> ("Output Current"=→"Output Voltage":dbl)  [unwired: 11 in, 2 out]
      n140 = call-poly <vilib>:"CTRE_Phoenix_MotorController_Get_Enhanced.vi"("PhoenixMotorControlDevRef"=w295, "error in"=w294) -> ("Output Current"=→"Output Voltage 2":dbl)  [unwired: 11 in, 2 out]
      n141 = call <vilib>:"CTRE_Phoenix_MotorControl_RefNumRegistryGet.vi"("refnum name"="frontRight") -> ("error out"=w291:errorcluster, "PhoenixMotorControlDevRef"=w292:T5)  [unwired: 9 in]
      n142 = call <vilib>:"CTRE_Phoenix_MotorControl_RefNumRegistryGet.vi"("refnum name"="rearRight") -> ("error out"=w288:errorcluster, "PhoenixMotorControlDevRef"=w289:T5)  [unwired: 9 in]
      n143 = call-poly <vilib>:"CTRE_Phoenix_MotorController_Get_Enhanced.vi"("PhoenixMotorControlDevRef"=w292, "error in"=w291) -> ("Output Current"=→"Output Voltage 3":dbl)  [unwired: 11 in, 2 out]
      n144 = call-poly <vilib>:"CTRE_Phoenix_MotorController_Get_Enhanced.vi"("PhoenixMotorControlDevRef"=w289, "error in"=w288) -> ("Output Current"=→"Output Voltage 4":dbl)  [unwired: 11 in, 2 out]
    }
    frame Enabled {
    }
  }
